vi "Register Sessions.vi"(8 "error in":errorcluster, 11 "session reservation in":refnum<class "Session Reservation.lvclass">) -> (0 "error out":errorcluster, 3 "session reservation out":refnum<class "Session Reservation.lvclass">)   [LabVIEW 2021, in "NI Session Management V1 Client.lvlib" / "Session Reservation.lvclass"]
doc: "Registers sessions with the session management service for shared use."
uses:
  Session Reservation.lvclass
  Session Reservation.lvclass/Session Reservation.ctl
  gRPC/Generated APIs/ni/measurementlink/sessionmanagement/v1/RPC Messages/ni_measurementlink_sessionmanagement_v1_ChannelMapping.ctl
  gRPC/Generated APIs/ni/measurementlink/sessionmanagement/v1/ni.measurementlink.sessionmanagement.v1.api.lvlib
  gRPC/Generated APIs/ni/measurementlink/sessionmanagement/v1/RPC Messages/nidevice_grpc_Session.ctl
  gRPC/Generated APIs/ni/measurementlink/sessionmanagement/v1/RPC Messages/ni_measurementlink_sessionmanagement_v1_SessionInformation.ctl
  gRPC/Generated APIs/ni/measurementlink/sessionmanagement/v1/RPC Messages/ni_measurementlink_sessionmanagement_v1_RegisterSessionsRequest.ctl
  gRPC/Generated APIs/ni/measurementlink/sessionmanagement/v1/RPC Messages/ni_measurementlink_sessionmanagement_v1_SessionInformation_AnnotationsEntry.ctl
  bb748151-28a4-4a68-b179-b8173ff3c443.vi
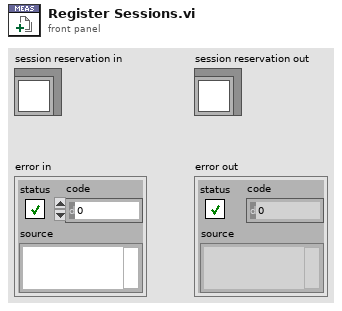
[diagram p1: front panel]
types:
  T1 = typedef "ni.measurementlink.sessionmanagement.v1.api.lvlib/ni_measurementlink_sessionmanagement_v1_SessionInformation_AnnotationsEntry.ctl" = cluster{"key":string, "value":string}
  T2 = typedef "ni.measurementlink.sessionmanagement.v1.api.lvlib/ni_measurementlink_sessionmanagement_v1_RegisterSessionsRequest.ctl" = cluster{"sessions":T3[]}
  T3 = typedef "ni.measurementlink.sessionmanagement.v1.api.lvlib/ni_measurementlink_sessionmanagement_v1_SessionInformation.ctl" = cluster{"session":T4, "resource_name":string, "channel_list":string, "instrument_type_id":string, "session_exists":bool, "session_reserved":bool, "channel_mappings":T5[], "annotations":T1[]}
  T4 = typedef "ni.measurementlink.sessionmanagement.v1.api.lvlib/nidevice_grpc_Session.ctl" = cluster{"name":string}
  T5 = typedef "ni.measurementlink.sessionmanagement.v1.api.lvlib/ni_measurementlink_sessionmanagement_v1_ChannelMapping.ctl" = cluster{"pin_or_relay_name":string, "site":i32, "channel":string, "multiplexer_resource_name":string, "multiplexer_route":string}
  T6 = typedef "NI Session Management V1 Client.lvlib/Session Reservation.lvclass/Data.ctl" = cluster{"session and driver infos":T7[], "pin or relay names":string[], "connection map":refnum<class "Connection Map.lvclass">, "pin map context":T9, "reservation observer":refnum<class "IReservation Observer.lvclass">, "dvr valid":bool, "group mappings":T10}
  T7 = typedef "NI Session Management V1 Client.lvlib/Session Reservation.lvclass/Session and Driver Info.ctl" = cluster{"session info":T3, "session":variant, "session factory":refnum<class "ISession Factory.lvclass">, "initialize and close session behavior":T8}
  T8 = typedef "NI Session Management Instrument.lvlib/ISession Factory.lvclass/Initialize and Close Session Behavior.ctl" = enum16{"Initialize and Close", "Attach and Detach", "Initialize and Detach", "Attach and Close"}
  T9 = typedef "ni.measurementlink.sessionmanagement.v1.api.lvlib/ni_measurementlink_PinMapContext.ctl" = cluster{"pin_map_id":string, "sites":i32[]}
  T10 = typedef "NI Session Management V1 Client.lvlib/Session Reservation.lvclass/Group Mapping.ctl" = map{string, string[]}
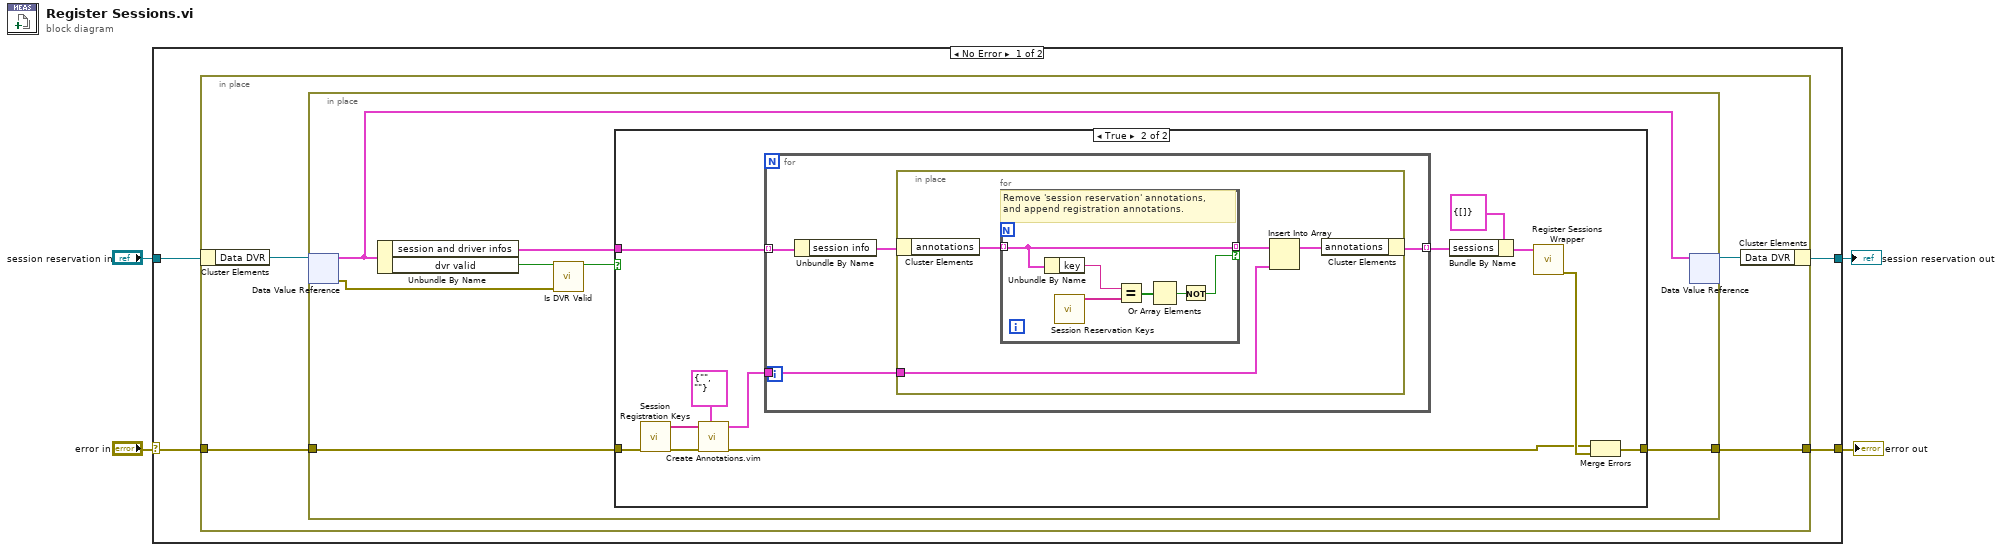
[diagram p0: block diagram]
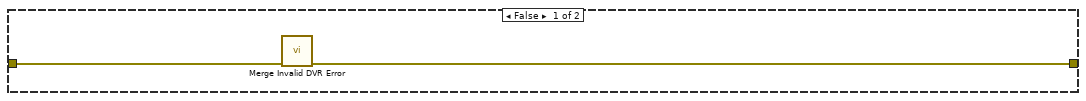
[diagram p2: hidden frame]
diagram:
  n1 = case shown="No Error" "error in" {
    selector: "error in" -> [w6 w47]
    tunnel: [w7 w48] -> w2
    tunnel: "session reservation in" -> [w8 w48]
    tunnel: [w5 w47] -> w1
    frame No Error {
      n2 = in-place {
        in-place-border: w6 -> [w10]
        in-place-border: [w9] -> w5
        n3 = in-place-cluster #1(w8) -> ("Data DVR"=w12:refnum<data-value>)
        n4 = in-place {
          in-place-border: w10 -> [w15]
          in-place-border: [w14] -> w9
          n5 = in-place-dvr #2(w12) -> (w13:T6, w18:errorcluster)
          n6 = Unbundle By Name(w13) -> ("session and driver infos"=w16:T7[], "dvr valid"=w19:bool)
          n7 = call "Is DVR Valid.vi"("dvr error in"=w18, "dvr valid in"=w19) -> ("dvr valid out"=w17:bool)  [unwired: 9 in]
          n8 = case shown="True" w17 {
            tunnel: w16 -> [_ w28]
            tunnel: w15 -> [w21 w26]
            tunnel: [w20 w31] -> w14
            frame False {
              n9 = call "Merge Invalid DVR Error.vi"("error in"=w21) -> ("error out"=w20:errorcluster)  [unwired: 10 in]
            }
            frame True {
              n10 = call "Session Registration Keys.vi"() -> ("register annotation keys"=w23:string[])  [unwired: 11 in]
              n11 = call "Create Annotations.vim"("annotation typedef"=T1 {"key"="", "value"=""} ("ni_measurementlink_sessionmanagement_v1_SessionInformation_AnnotationsEntry"), "error in"=w26, "annotation keys"=w23) -> ("error out"=w25:errorcluster, "annotations array"=w24:T1[])  [unwired: 7 in]
              n12 = for {
                tunnel: w28 -> [w36] mode=indexing
                tunnel: [w34] -> w27 mode=indexing
                tunnel: w24 -> [w33]
                n13 = Unbundle By Name(w36) -> ("session info"=w35:T3)
                n14 = in-place {
                  in-place-border: w33 -> [w38]
                  n15 = in-place-cluster #3(w35) -> ("annotations"=w37:T1[])
                  n16 = for {
                    tunnel: [w43] -> w39 mode=indexing if=w44
                    tunnel: w37 -> [w43] mode=indexing
                    # "Remove 'session reservation' annotations,\nand append registration annotations."
                    n17 = Unbundle By Name(w43) -> ("key"=w41:string)
                    n18 = call "Session Reservation Keys.vi"() -> ("reserve annotation keys"=w42:string[])  [unwired: 11 in]
                    n19 = Equal?(x=w41, y=w42) -> (x = y?=w45:bool[])
                    n20 = Or Array Elements(Boolean array=w45) -> (logical OR=w46:bool)
                    n21 = Not(x=w46) -> (.not. x?=w44:bool)
                  }
                  n22 = Insert Into Array(array=w39, new element=w38) -> (w40:T1[])  [unwired: 1 in]
                  n23 = in-place-cluster #3("annotations"=w40) -> (w34:T3)
                }
              }
              n24 = Bundle By Name(cluster=T2 {"sessions"=[]} ("Request Data"), "sessions"=w27) -> (w30:T2)
              n25 = call "Register Sessions Wrapper.vi"("request data"=w30) -> ("error out"=w29:errorcluster)  [unwired: 9 in, 1 out]
              n26 = Merge Errors(w25, w29) -> (w31:errorcluster)
            }
          }
          n27 = in-place-dvr #2(w13) -> (w11:refnum<data-value>)  [unwired: 1 out]
        }
        n28 = in-place-cluster #1("Data DVR"=w11) -> (w7:refnum<class "Session Reservation.lvclass">)
      }
    }
    frame Error {
    }
  }
  "error out" <- w1
  "session reservation out" <- w2
